vi "DAC Run.vi"(8 "error in":errorcluster, 11 "DAC HMP4040 in":refnum<class "DAC HMP4040.lvclass">) -> (0 "error out":errorcluster, 3 "DAC HMP4040 out":refnum<class "DAC HMP4040.lvclass">)   [LabVIEW 2019, in "DAC.lvlib" / "DAC HMP4040.lvclass"]
uses:
  DAC HMP4040.lvclass
  DAC.lvclass
  Results/Results Method.ctl
  Results/Results.lvlib
  Results/Heat Flow Results/Heat Flow Results.lvclass
  C:/Users/krio/Documents/LV_Projects/test-stand/App/DAC/DAC.lvclass
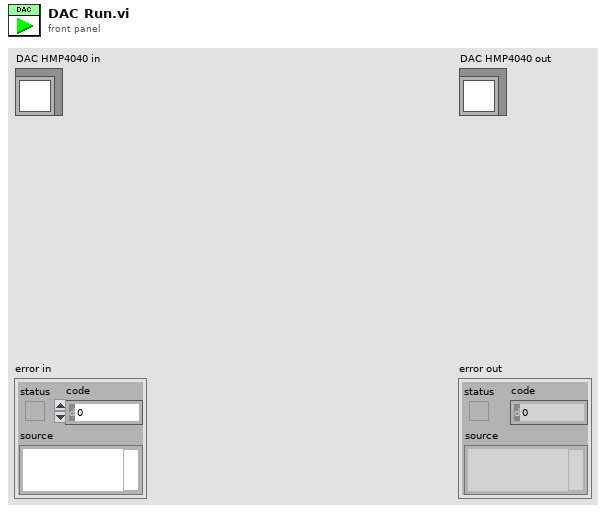
[diagram p1: front panel]
types:
  T1 = typedef "Results.lvlib/Results Method.ctl" = enum16{"Get", "Set"}
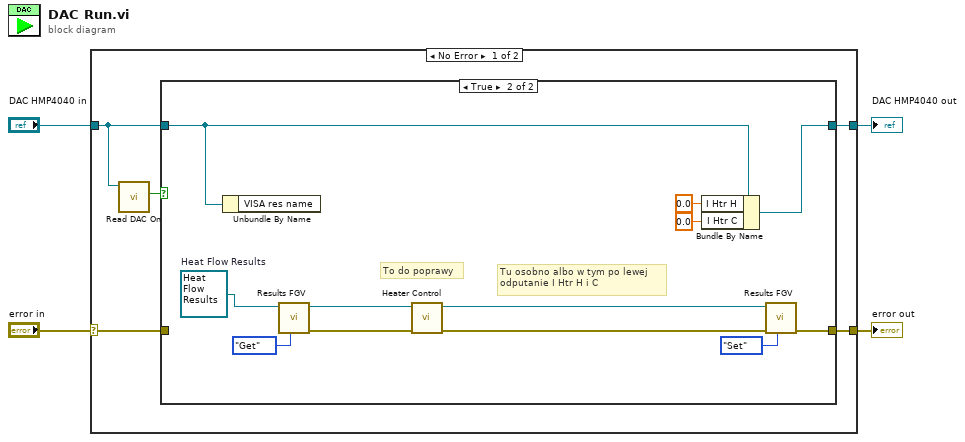
[diagram p0: block diagram]
diagram:
  n1 = case shown="No Error" "error in" {
    selector: "error in" -> [w7 w25]
    tunnel: [w6 w25] -> w2
    tunnel: [w8 w24] -> w1
    tunnel: "DAC HMP4040 in" -> [w5 w24]
    frame No Error {
      n2 = call "Read DAC On.vi"("DAC in"=w5) -> ("DAC On"=w9:bool)  [unwired: 8 in, 2 out]
      n3 = case shown="True" w9 {
        tunnel: w5 -> [w11 w23]
        tunnel: [w11 w20] -> w8
        tunnel: w7 -> [w10 _]
        tunnel: [w10 w19] -> w6
        frame False {
        }
        frame True {
          w18 = refnum<class "Heat Flow Results.lvclass"> refnum  # Heat Flow Results
          # "Tu osobno albo w tym po lewej\nodputanie I Htr H i C"
          # "To do poprawy"
          n4 = Unbundle By Name(w23) -> ()  [unwired: 1 out]
          n5 = call-dynamic "Results FGV.vi"("Method"=Results_Method."Get", "Results in"=w18) -> ("error out"=w13:errorcluster, "Results out"=w15:refnum<class "Heat Flow Results.lvclass">)  [unwired: 8 in]
          n6 = call "Heater Control.vi"("error in"=w13, "HeatFlow Results in"=w15) -> ("error out"=w12:errorcluster, "HeatFlow Results out"=w14:refnum<class "Heat Flow Results.lvclass">)  [unwired: 6 in, 2 out]
          n7 = Bundle By Name(cluster=w23, "I Htr H"=0.0, "I Htr C"=0.0) -> (w20:refnum<class "DAC HMP4040.lvclass">)
          n8 = call-dynamic "Results FGV.vi"("Method"=Results_Method."Set", "error in"=w12, "Results in"=w14) -> ("error out"=w19:errorcluster)  [unwired: 7 in, 1 out]
        }
      }
    }
    frame Error {
    }
  }
  "error out" <- w2
  "DAC HMP4040 out" <- w1
